vi "Autonomous Independent.vi"   [LabVIEW 2014]
doc: "This VI is called when autonomous begins, and will automatically be terminated when autonomous ends. You can carry out timed or sensor driven robot movement independently without needing to return to the caller."
uses:
  <vilib>/Rock Robotics/WPI/Joystick/WPI_JoystickGetSetRefNum.vi
  <vilib>/Rock Robotics/Network Tables/SD Write Numeric Array.vi
  <vilib>/Rock Robotics/WPI/RobotDrive/WPI_RobotDriveGetSetRefNum.vi
  <vilib>/Rock Robotics/WPI/RobotDrive/WPI_RobotDriveMecanumDrive_Cartesian.vi
types:
  T1 = typedef "WPI_JoystickDevRef.ctl" = cluster{"Device":T2}
  T2 = typedef "WPI_JoystickDeviceEnum.ctl" = enum16{"USB 0", "USB 1", "USB 2", "USB 3", "USB 4", "USB 5"}
  T3 = typedef "WPI_DigitalInputDevRef.ctl" = cluster{"DevStatus":errorcluster, "DIO Channel":T4, "Controller":T5}
  T4 = typedef "FPGA_DIOChannel.ctl" = enum8{"DIO 0", "DIO 1", "DIO 2", "DIO 3", "DIO 4", "DIO 5", "DIO 6", "DIO 7", "DIO 8", "DIO 9", "DIO MXP 0", "DIO MXP 1", "DIO MXP 2", "DIO MXP 3", "DIO MXP 4", "DIO MXP 5", "DIO MXP 6", "DIO MXP 7", "DIO MXP 8", "DIO MXP 9", "DIO MXP 10", "DIO MXP 11", "DIO MXP 12", "DIO MXP 13", "DIO MXP 14", "DIO MXP 15", "Invalid"}
  T5 = typedef "FPGA_TypedefDigitalModule.ctl" = enum16{"Controller 1"}
  T6 = typedef "WPI_MotorControlDeviceRef.ctl" = cluster{"DeviceStatus":errorcluster, "Type":T7, "PWM":cluster{"Controller":T5, "PWM Channel":T8, "DeadBand":T9}, "CAN":cluster{"Device Number":u8, "Control Mode":T10, "Semaphore":T11, "Max Vout":dbl, "TalonSRX Control Mode":T12}, "Invert":bool, "TransformRef":T13, "InvTransformRef":T13}
  T7 = typedef "WPI_MotorControlType.ctl" = enum16{"PWM", "CAN", "CANTalonSRX"}
  T8 = typedef "FPGA_DIOPWMChannel.ctl" = enum8{"PWM 0", "PWM 1", "PWM 2", "PWM 3", "PWM 4", "PWM 5", "PWM 6", "PWM 7", "PWM 8", "PWM 9", "PWM MXP 0", "PWM MXP 1", "PWM MXP 2", "PWM MXP 3", "PWM MXP 4", "PWM MXP 5", "PWM MXP 6", "PWM MXP 7", "PWM MXP 8", "PWM MXP 9", "Invalid"}
  T9 = typedef "WPI_PWMDeadband.ctl" = cluster{"Name":string, "maxPositivePwm":i32, "minPositivePwm":i32, "centerPwm":i32, "maxNegativePwm":i32, "minNegativePwm":i32, "angularRange":u16}
  T10 = typedef "WPI_CANJaguar_ControlMode.ctl" = enum8{"Percent VBus", "Current", "Speed", "Position", "Voltage"}
  T11 = typedef "Semaphore RefNum" = refnum<k1>
  T12 = typedef "WPI_CANTalonSRX_APIControlMode.ctl" = enum8{"Percent VBus", "Speed", "Position", "Slave", "Unchanged / Invalid"}
  T13 = typedef "WPI_PWMTransform_ConPane.ctl" = refnum<vi>
  T14 = typedef "WPI_RobotDriveDevRef.ctl" = cluster{"DevStatus":errorcluster, "Motors[]":T6[], "Square Inputs":bool, "Max Output":dbl}
  T15 = typedef "WPI_CANTalonSRX_GlobalStatus.ctl" = cluster{"Applied Throttle":dbl, "Module Enabled":bool, "CAN Error":errorcluster, "Closed Loop Error":dbl, "Forward Limit Switch Closed":bool, "Reverse Limit Switch Closed":bool, "Sensor Position":dbl, "Sensor Velocity":dbl, "Current":dbl, "Sticky Fault - Over Temp":bool, "Sticky Fault - Under Voltage":bool, "Sticky Fault - Forward Limit":bool, "Sticky Fault - Reverse Limit":bool, "Sticky Fault - Forward Soft Limit":bool, "Sticky Fault - Reverse Soft Limit":bool, "Brake is Enabled":bool, "Encoder Position":dbl, "Encoder Velocity":dbl, "Encoder Index Count":dbl, "Encoder A Pin State":bool, "Encoder B Pin State":bool, "Encoder Index Pin State":bool, "Analog In":dbl, "Analog In Velocity":dbl, "Temperature (C)":dbl, "Battery Voltage":dbl}
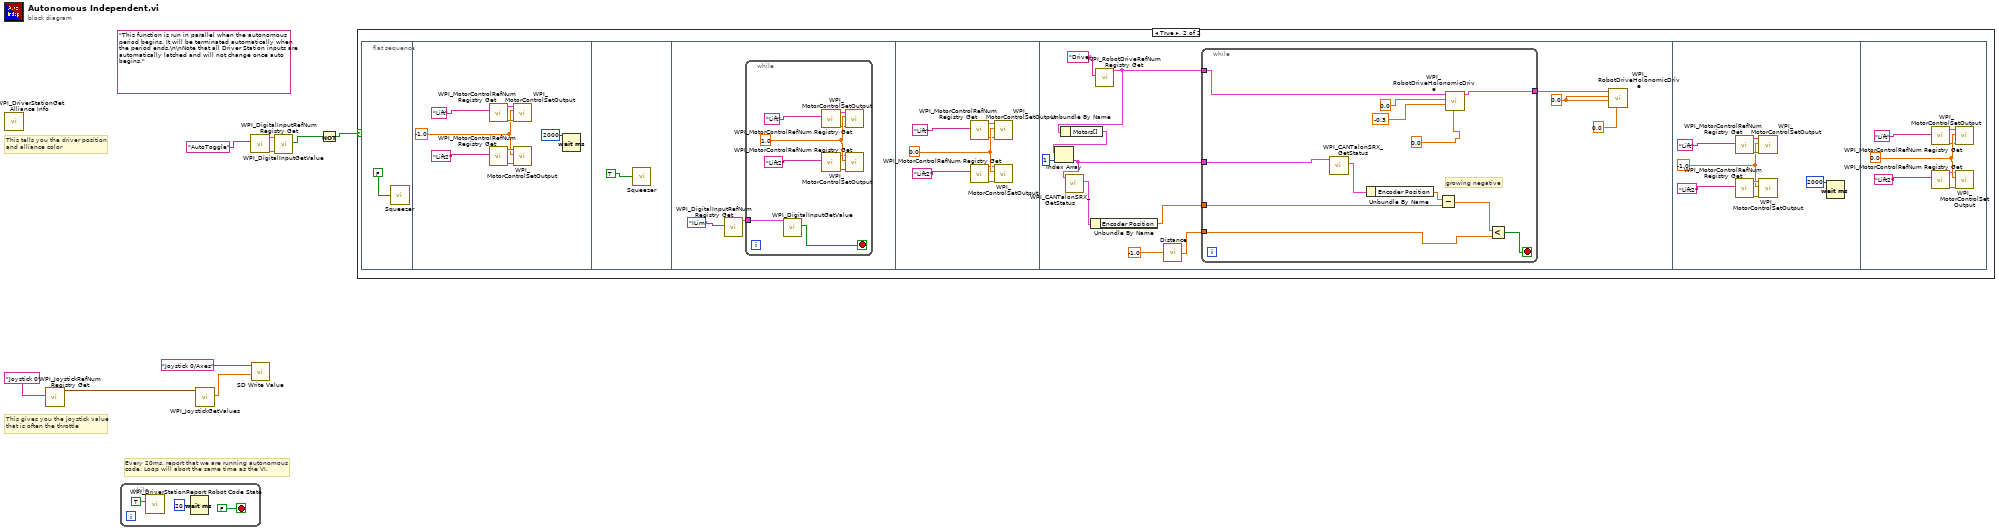
[diagram p0: block diagram]
diagram:
  (unwired) "This function is run in parallel when the autonomous period begins. It will be terminated automatically when the period ends.\n\nNote that all Driver Station inputs are automatically latched and will not change once auto begins."
  # "Every 20ms, report that we are running autonomous\ncode. Loop will abort the same time as the VI."
  # "This gives you the joystick value\nthat is often the throttle"
  # "This tells you the driver position\nand alliance color"
  n1 = call <vilib>:"WPI_DriverStationGet Alliance Info.vi"() -> ()  [unwired: 12 out]
  n2 = call <vilib>:"WPI_JoystickRefNum Registry Get.vi"("refnum name"="Joystick 0") -> ("JoystickDevRef"=w8:T1)  [unwired: 1 in, 9 out]
  n3 = while {
    stop <- FALSE stop-if-true
    n4 = call <vilib>:"WPI_DriverStationReport Robot Code State.vi"("Autonomous"=TRUE) -> ()  [unwired: 10 in, 1 out]
    n5 = Wait (ms)(milliseconds to wait=u32 20) -> ()  [unwired: 1 out]
  }
  n6 = call <vilib>:"WPI_JoystickGetValues.vi"("JoystickDevRef"=w8) -> ("Axes"=w6:dbl[])  [unwired: 6 in, 4 out]
  n7 = call <vilib>:"WPI_DigitalInputRefNum Registry Get.vi"("refnum name"="AutoToggle") -> ("error out"=w5:errorcluster, "DigitalInputDevRef"=w4:T3)  [unwired: 9 in]
  n8 = call-poly <vilib>:"SD Write Value.vi"("Numeric Array"=w6, "Name"="Joystick 0/Axes") -> ()  [unwired: 8 in, 2 out]
  n9 = call <vilib>:"WPI_DigitalInputGetValue.vi"("error in (no error)"=w5, "DigitalInputDevRef"=w4) -> ("Value"=w2:bool)  [unwired: 7 in, 2 out]
  n10 = Not(x=w2) -> (.not. x?=w1:bool)
  n11 = case shown="True" w1 {
    frame False {
    }
    frame True {
      n12 = flat-sequence {
        frame #0 {
          n13 = call "Squeezer.vi"("Direction"=FALSE) -> ()
        }
        frame #1 {
          w14 = -1.0
          n14 = call <vilib>:"WPI_MotorControlRefNum Registry Get.vi"("refnum name"="Lift") -> ("error out"=w19:errorcluster, "MotorControlDevRef"=w18:T6)  [unwired: 9 in]
          n15 = call <vilib>:"WPI_MotorControlRefNum Registry Get.vi"("refnum name"="Lift2") -> ("error out"=w16:errorcluster, "MotorControlDevRef"=w15:T6)  [unwired: 9 in]
          n16 = call <vilib>:"WPI_MotorControlSetOutput.vi"("error in (no error)"=w19, "Output"=w14, "MotorControlDevRef"=w18) -> ()  [unwired: 6 in, 3 out]
          n17 = call <vilib>:"WPI_MotorControlSetOutput.vi"("error in (no error)"=w16, "Output"=w14, "MotorControlDevRef"=w15) -> ()  [unwired: 6 in, 3 out]
          n18 = Wait (ms)(milliseconds to wait=2000) -> ()  [unwired: 1 out]
        }
        frame #2 {
          n19 = call "Squeezer.vi"("Direction"=TRUE) -> ()
        }
        frame #3 {
          n20 = call <vilib>:"WPI_DigitalInputRefNum Registry Get.vi"("refnum name"="ILim") -> ("DigitalInputDevRef"=w23:T3)  [unwired: 9 in, 1 out]
          n21 = while {
            tunnel: w23 -> [w33]
            stop <- w32 stop-if-true
            w31 = 1.0
            n22 = call <vilib>:"WPI_DigitalInputGetValue.vi"("DigitalInputDevRef"=w33) -> ("Value"=w32:bool)  [unwired: 8 in, 2 out]
            n23 = call <vilib>:"WPI_MotorControlRefNum Registry Get.vi"("refnum name"="Lift") -> ("error out"=w26:errorcluster, "MotorControlDevRef"=w27:T6)  [unwired: 9 in]
            n24 = call <vilib>:"WPI_MotorControlRefNum Registry Get.vi"("refnum name"="Lift2") -> ("error out"=w29:errorcluster, "MotorControlDevRef"=w30:T6)  [unwired: 9 in]
            n25 = call <vilib>:"WPI_MotorControlSetOutput.vi"("error in (no error)"=w26, "Output"=w31, "MotorControlDevRef"=w27) -> ()  [unwired: 6 in, 3 out]
            n26 = call <vilib>:"WPI_MotorControlSetOutput.vi"("error in (no error)"=w29, "Output"=w31, "MotorControlDevRef"=w30) -> ()  [unwired: 6 in, 3 out]
          }
        }
        frame #4 {
          w40 = 0.0
          n27 = call <vilib>:"WPI_MotorControlRefNum Registry Get.vi"("refnum name"="Lift") -> ("error out"=w35:errorcluster, "MotorControlDevRef"=w36:T6)  [unwired: 9 in]
          n28 = call <vilib>:"WPI_MotorControlRefNum Registry Get.vi"("refnum name"="Lift2") -> ("error out"=w38:errorcluster, "MotorControlDevRef"=w39:T6)  [unwired: 9 in]
          n29 = call <vilib>:"WPI_MotorControlSetOutput.vi"("error in (no error)"=w35, "Output"=w40, "MotorControlDevRef"=w36) -> ()  [unwired: 6 in, 3 out]
          n30 = call <vilib>:"WPI_MotorControlSetOutput.vi"("error in (no error)"=w38, "Output"=w40, "MotorControlDevRef"=w39) -> ()  [unwired: 6 in, 3 out]
        }
        frame #5 {
          w42 = 0.0 ("X")
          n31 = call <vilib>:"WPI_RobotDriveRefNum Registry Get.vi"("refnum name"="Drive") -> ("RobotDriveDevRef"=w48:T14)  [unwired: 9 in, 1 out]
          n32 = Unbundle By Name(w48) -> ("Motors[]"=w50:T6[])
          n33 = Index Array(array=w50, index=1) -> (element=w43:T6)
          n34 = call <vilib>:"WPI_CANTalonSRX_GetStatus.vi"("CAN Talon SRX Ref"=w43) -> ("Talon SRX Status"=w49:T15)  [unwired: 8 in, 2 out]
          n35 = Unbundle By Name(w49) -> ("Encoder Position"=w47:dbl)
          n36 = call "Distance.vi"("Feet"=-1.0) -> ("Distance"=w45:dbl)
          n37 = while {
            tunnel: w48 -> [w62]
            tunnel: [w60] -> w52
            tunnel: w47 -> [w57]
            tunnel: w45 -> [w55]
            tunnel: w43 -> [w54]
            stop <- w59 stop-if-true
            # "growing negative"
            n38 = call <vilib>:"WPI_CANTalonSRX_GetStatus.vi"("CAN Talon SRX Ref"=w54) -> ("Talon SRX Status"=w61:T15)  [unwired: 8 in, 2 out]
            n39 = Unbundle By Name(w61) -> ("Encoder Position"=w58:dbl)
            n40 = Subtract(x=w58, y=w57) -> (x-y=w56:dbl)
            n41 = call-poly <vilib>:"WPI_RobotDriveHolonomicDrive.vi"("Rotation"=0.0, "Y"=-0.3, "X"=0.0, "RobotDriveDevRef"=w62) -> ("RobotDriveDevRef"=w60:T14)  [unwired: 5 in, 2 out]
            n42 = Less?(x=w56, y=w55) -> (x < y?=w59:bool)
          }
          n43 = call-poly <vilib>:"WPI_RobotDriveHolonomicDrive.vi"("Rotation"=0.0, "Y"=w42, "X"=w42, "RobotDriveDevRef"=w52) -> ()  [unwired: 5 in, 3 out]
        }
        frame #6 {
          w65 = -1.0
          n44 = call <vilib>:"WPI_MotorControlRefNum Registry Get.vi"("refnum name"="Lift") -> ("error out"=w70:errorcluster, "MotorControlDevRef"=w69:T6)  [unwired: 9 in]
          n45 = call <vilib>:"WPI_MotorControlRefNum Registry Get.vi"("refnum name"="Lift2") -> ("error out"=w67:errorcluster, "MotorControlDevRef"=w66:T6)  [unwired: 9 in]
          n46 = call <vilib>:"WPI_MotorControlSetOutput.vi"("error in (no error)"=w70, "Output"=w65, "MotorControlDevRef"=w69) -> ()  [unwired: 6 in, 3 out]
          n47 = call <vilib>:"WPI_MotorControlSetOutput.vi"("error in (no error)"=w67, "Output"=w65, "MotorControlDevRef"=w66) -> ()  [unwired: 6 in, 3 out]
          n48 = Wait (ms)(milliseconds to wait=2000) -> ()  [unwired: 1 out]
        }
        frame #7 {
          w79 = 0.0
          n49 = call <vilib>:"WPI_MotorControlRefNum Registry Get.vi"("refnum name"="Lift") -> ("error out"=w74:errorcluster, "MotorControlDevRef"=w75:T6)  [unwired: 9 in]
          n50 = call <vilib>:"WPI_MotorControlRefNum Registry Get.vi"("refnum name"="Lift2") -> ("error out"=w77:errorcluster, "MotorControlDevRef"=w78:T6)  [unwired: 9 in]
          n51 = call <vilib>:"WPI_MotorControlSetOutput.vi"("error in (no error)"=w74, "Output"=w79, "MotorControlDevRef"=w75) -> ()  [unwired: 6 in, 3 out]
          n52 = call <vilib>:"WPI_MotorControlSetOutput.vi"("error in (no error)"=w77, "Output"=w79, "MotorControlDevRef"=w78) -> ()  [unwired: 6 in, 3 out]
        }
      }
    }
  }
